vi "Function_Generator_Ex.vi"() -> ()   [LabVIEW 2026]
panel:
  out "Pict Ring":u16(ring)
  out "Stop":bool
  in  "Duty":u8 max=100
  in  "Frecuencia (Hz)":dbl=0.001 min=0.001 max=2000.0
  in  "Offset":dbl=0.001 min=0.0 max=3.3
  in  "Amplitud":dbl=0.001 min=0.0 max=3.3
  in  "Tipo de Onda":u16(ring) items=["Senoidal", "Triangular", "Cuadrada", "Sierra"]
  in  "Canal":u8
  out "Status":string
  in  "VISA resource name":refnum<visa-resource-name>
  in  "Stop Button":bool
  out "error out":errorcluster
  # "Ejemplo: Generador de funciones"
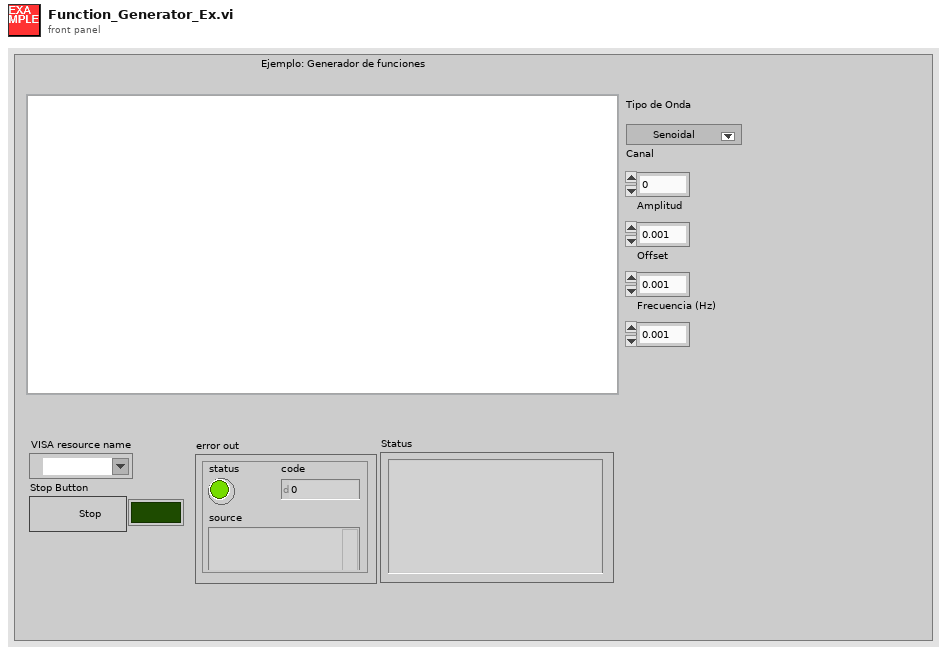
[diagram p1: front panel]
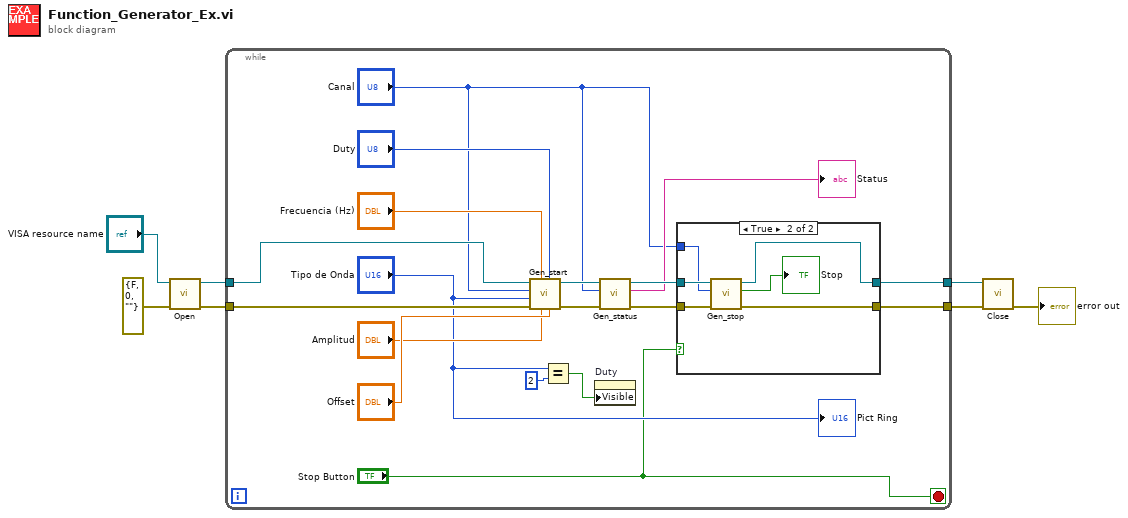
[diagram p0: block diagram]
diagram:
  n1 = call "Open.vi"("error in (no error)"=errorcluster {"status"=FALSE, "code"=0, "source"=""}, "VISA resource name"="VISA resource name") -> ("error out"=w7:errorcluster, "VISA resource name out"=w6:refnum<visa-resource-name>)  [unwired: 8 in]
  n2 = while {
    tunnel: w6 -> [w25]
    tunnel: w7 -> [w24]
    tunnel: [w21] -> w2
    tunnel: [w18] -> w1
    stop <- "Stop Button" stop-if-true
    n3 = call "Gen_start.vi"("Offset"="Offset", "Duty"="Duty", "Amplitud"="Amplitud", "Frecuencia (Hz)"="Frecuencia (Hz)", "error in (no error)"=w24, "Tipo de Onda"="Tipo de Onda", "Canal"="Canal", "VISA resource name"=w25) -> ("error out"=w22:errorcluster, "VISA resource name out"=w23:refnum<visa-resource-name>)  [unwired: 1 in, 1 out]
    n4 = Equal?(x="Tipo de Onda", y=u16 2) -> (x = y?=w10:bool)
    n5 = property on="Duty" class="DigNum (strict)"("Visible"=w10) -> ()  [unwired: 2 in, 2 out]
    n6 = call "Gen_status.vi"("error in (no error)"=w22, "Canal"="Canal", "VISA resource name"=w23) -> ("error out"=w19:errorcluster, "respuesta"=→"Status":string, "VISA resource name out"=w20:refnum<visa-resource-name>)  [unwired: 6 in]
    n7 = case shown="True" "Stop Button" {
      tunnel: [w27 w30] -> w21
      tunnel: w20 -> [w27 w33]
      tunnel: w19 -> [w26 w32]
      tunnel: [w26 w31] -> w18
      tunnel: "Canal" -> [_ w28]
      frame False {
      }
      frame True {
        n8 = call "Gen_stop.vi"("error in (no error)"=w32, "Canal"=w28, "VISA resource name"=w33) -> ("error out"=w31:errorcluster, "ok"=→"Stop":bool, "VISA resource name out"=w30:refnum<visa-resource-name>)  [unwired: 6 in]
      }
    }
    "Pict Ring" <- "Tipo de Onda"
  }
  n9 = call "Close.vi"("error in (no error)"=w1, "VISA resource name"=w2) -> ("error out"=→"error out":errorcluster)  [unwired: 9 in]
